vi "UE_Cycle_Event_Duration.vi"(1 "start_ms":dbl, 2 "end_ms":dbl) -> (0 "duration_ms":dbl)   [LabVIEW 2026]
doc: "INTENT: Compute feedback-event duration in milliseconds from a shared monotonic clock. INPUTS: end_ms (double), start_ms (double). OUTPUTS: duration_ms (double). DESIGN CONSTRAINT: Used for TPL lift/lower cycle time; does not detect events. REQUIREMENTS: SRS-F-006. No physical hardware side effects. Acceptance requires native LabVIEW compilation and behavioral testing."
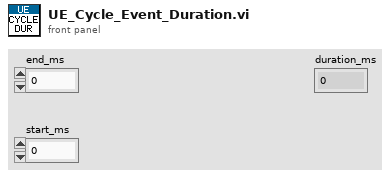
[diagram p1: front panel]
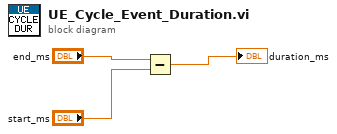
[diagram p0: block diagram]
diagram:
  n1 = Subtract(x="end_ms", y="start_ms") -> (x-y=→"duration_ms":dbl)
